vi "Offset Measurement Result.vi"(8 "error in (no error)":errorcluster, 9 "current offsets":dbl[](array[numeric]), 10 "Offset Measurement":T1={"phase"=enum."idle", "measureInputOffset"={"buffers"=0, "settle"=2, "timeout"=5.0, "channels"=[], "zero"=enum."both"}, "settle remaining"=0, "buffers remaining"=0, "deadline"=0, "sum"=[], "count"=0, "saved amplitudes"=[], "saved offsets"=[], "previous status"=enum."created"}, 11 "Instrument.DAQ in":refnum<class "Instrument.DAQ.lvclass">) -> (0 "error out":errorcluster, 1 "new offsets":dbl[](array[numeric]), 2 "Offset Measurement":T1={"phase"=enum."idle", "measureInputOffset"={"buffers"=0, "settle"=2, "timeout"=5.0, "channels"=[], "zero"=enum."both"}, "settle remaining"=0, "buffers remaining"=0, "deadline"=0, "sum"=[], "count"=0, "saved amplitudes"=[], "saved offsets"=[], "previous status"=enum."created"}, 3 "Instrument.DAQ out":refnum<class "Instrument.DAQ.lvclass">)   [LabVIEW 2019, in "Instrument.Lockin.lvlib" / "Instrument.DAQ.lvclass"]
uses:
  Instrument.DAQ.lvclass
  Typedefs/Offset Measurement--Cluster.ctl
  Lockin.Typedefs/API/Lockin.measureInputOffset Config--Cluster.ctl
  Lockin.Typedefs/API/Lockin.measureInputOffset.zero--enum.ctl
  Lockin.Typedefs/other/Status--enum.ctl
  Lockin.Typedefs/Lockin.Typedefs.lvlib
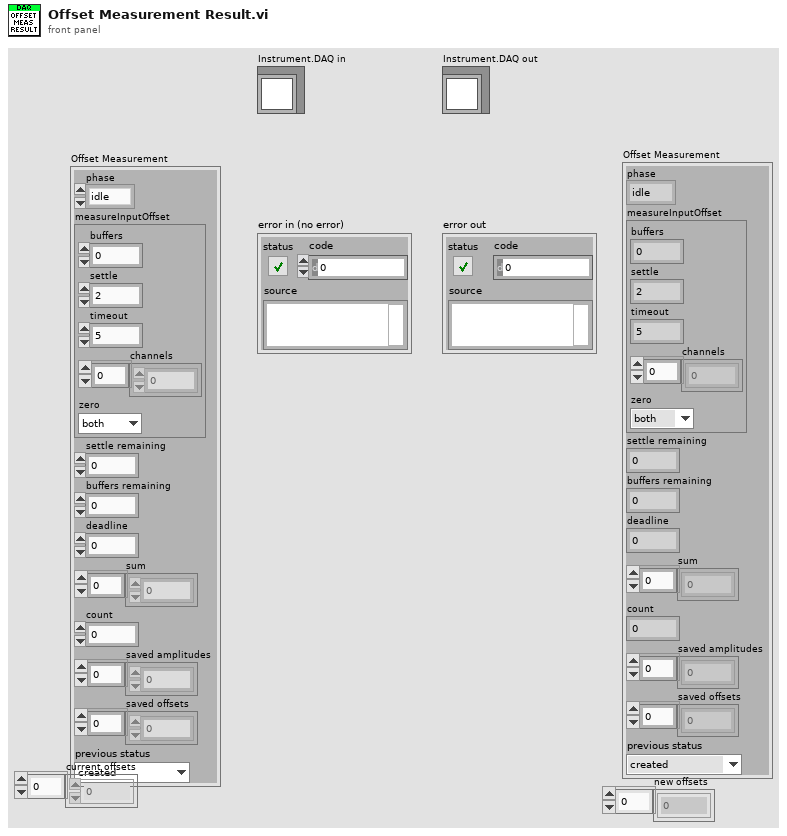
[diagram p1: front panel]
types:
  T1 = typedef "Instrument.Lockin.lvlib/Instrument.DAQ.lvclass/Offset Measurement--Cluster.ctl" = cluster{"phase":enum16{"idle", "zeroing", "settling", "averaging", "done", "aborted", "cancelled", "timed out"}, "measureInputOffset":T2, "settle remaining":i32, "buffers remaining":i32, "deadline":u32, "sum":dbl[], "count":i32, "saved amplitudes":dbl[], "saved offsets":dbl[], "previous status":T4}
  T2 = typedef "Lockin.Typedefs.lvlib/Lockin.measureInputOffset Config--Cluster.ctl" = cluster{"buffers":i32, "settle":i32, "timeout":dbl, "channels":i32[], "zero":T3}
  T3 = typedef "Lockin.Typedefs.lvlib/Lockin.measureInputOffset.zero--enum.ctl" = enum16{"both", "ac", "dc", "none"}
  T4 = typedef "Lockin.Typedefs.lvlib/Status--enum.ctl" = enum16{"idle", "created", "started", "stopped", "sweeping", "measuring offset"}
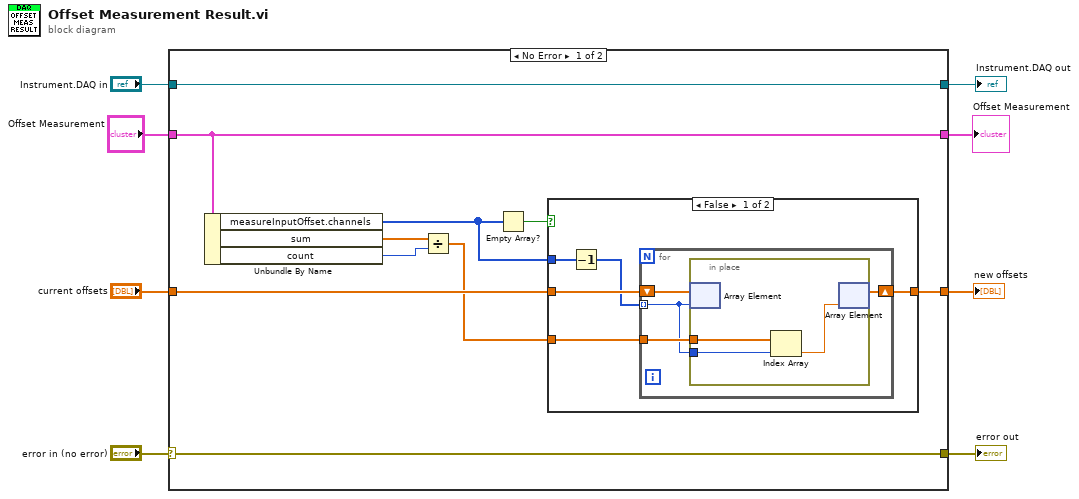
[diagram p0: block diagram]
diagram:
  n1 = case shown="No Error" "error in (no error)" {
    selector: "error in (no error)" -> [w18 w35]
    tunnel: "Offset Measurement" -> [w16 w33]
    tunnel: [w16 w33] -> w7
    tunnel: "current offsets" -> [w13 w32]
    tunnel: [w18 w35] -> w4
    tunnel: [w17 w34] -> w3
    tunnel: "Instrument.DAQ in" -> [w17 w34]
    tunnel: [w14 w32] -> w1
    frame No Error {
      n2 = Unbundle By Name(w16) -> ("measureInputOffset.channels"=w12:i32[], "sum"=w10:dbl[], "count"=w11:i32)
      n3 = Divide(x=w10, y=w11) -> (x/y=w9:dbl[])
      n4 = Empty Array?(array=w12) -> (empty?=w15:bool)
      n5 = case shown="False" w15 {
        tunnel: [w20 w31] -> w14
        tunnel: w9 -> [w19 w31]
        tunnel: w13 -> [w22 _]
        tunnel: w12 -> [w23 _]
        frame False {
          n6 = Decrement(x=w23) -> (x-1=w21:i32[])
          n7 = for {
            tunnel: w21 -> [w24] mode=indexing
            shift-right: [w26] -> w20
            shift-left: w22 -> [w27]
            tunnel: w19 -> [w25]
            n8 = in-place {
              in-place-border: w25 -> [w30]
              in-place-border: w24 -> [w29]
              n9 = in-place-array #1(w27, w24) -> ()  [unwired: 1 out]
              n10 = Index Array(array=w30, index=w29) -> (element=w28:dbl)
              n11 = in-place-array #1(w28) -> (w26:dbl[])  [unwired: 1 out]
            }
          }
        }
        frame True {
        }
      }
    }
    frame Error {
    }
  }
  "error out" <- w4
  "Instrument.DAQ out" <- w3
  "Offset Measurement" <- w7
  "new offsets" <- w1
